vi "LoadCFG.vi"(8 "error in (no error)":errorcluster, 11 "object in":refnum<class "DIO-Configuration.lvclass">) -> (0 "error out":errorcluster, 2 "Success?":bool, 3 "object out":refnum<class "DIO-Configuration.lvclass">)   [LabVIEW 2021, in "DIO-Configuration.lvclass"]
doc: "Loads Configuration"
uses:
  DIO-Configuration.lvclass
  C:/Users/averna/Documents/LV Gym DEMO/Factory Pattern/Generic Channel/Configuration/Configuration.lvclass
  Device Channels/DAQmx/DIO-Configuration_class/tdef/Direction.ctl
  DIO-Configuration.lvclass/DIO-Configuration.ctl
  Generic Channel/Configuration/properties/ReadConfigurationFile.vi
  <vilib>/Utility/config.llb/Read Key (String).vi
  Channels/DIO-Channel/DIO-Configuration_class/DIO-Configuration.lvclass
  <vilib>/Utility/config.llb/NI_LVConfig.lvlib
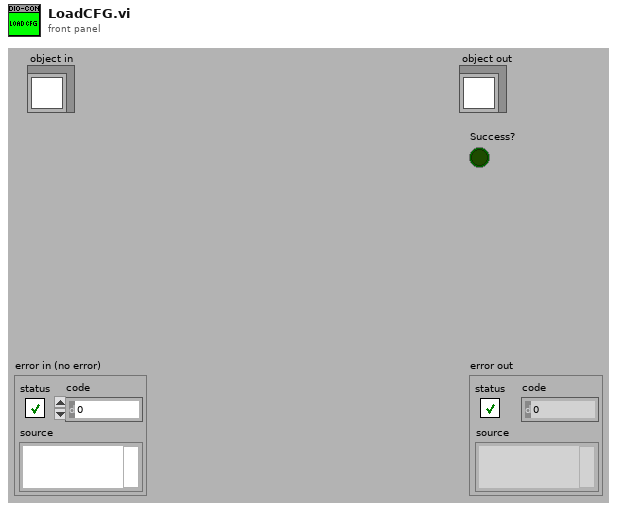
[diagram p1: front panel]
types:
  T1 = typedef "DIO-Configuration.lvclass/Direction.ctl" = enum16{"Input", "Output"}
  T2 = typedef "NI_LVConfig.lvlib/Config Data RefNum.ctl" = refnum<k1>
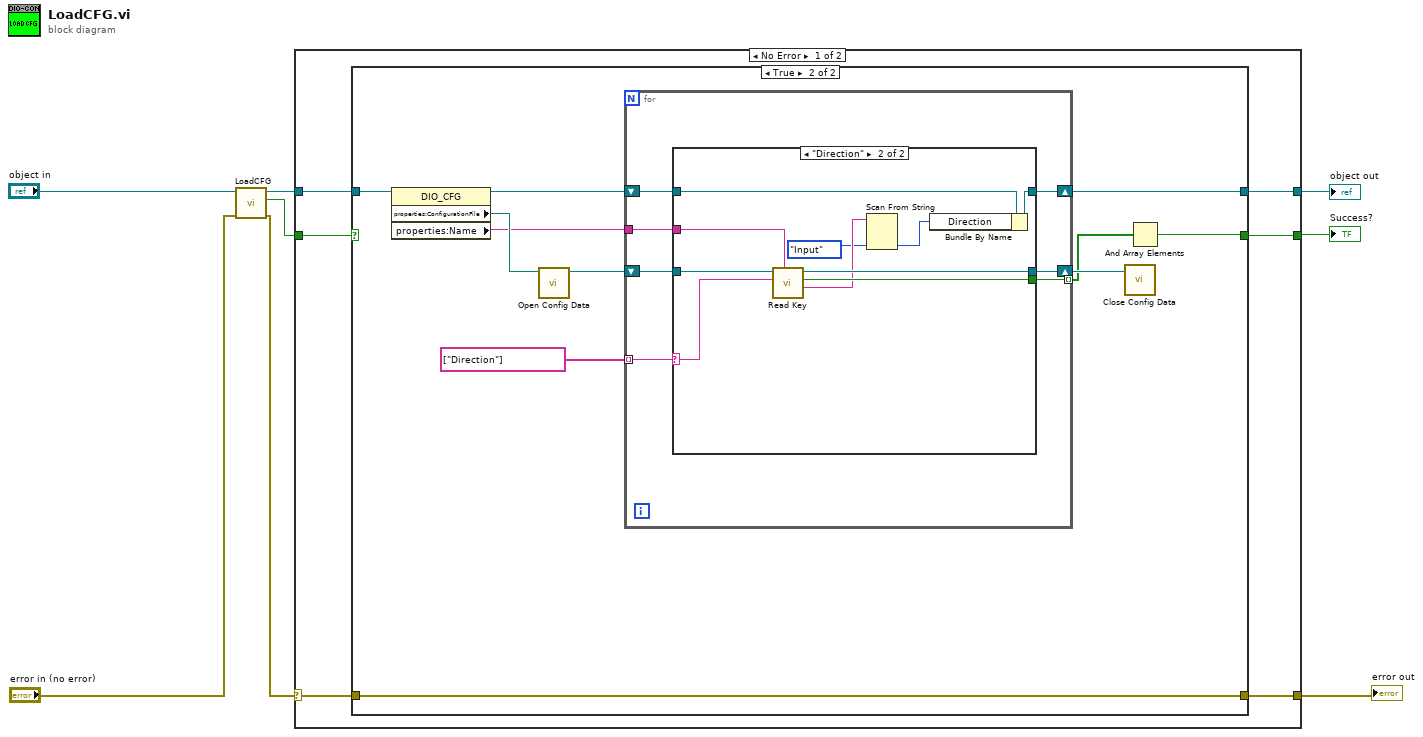
[diagram p0: block diagram]
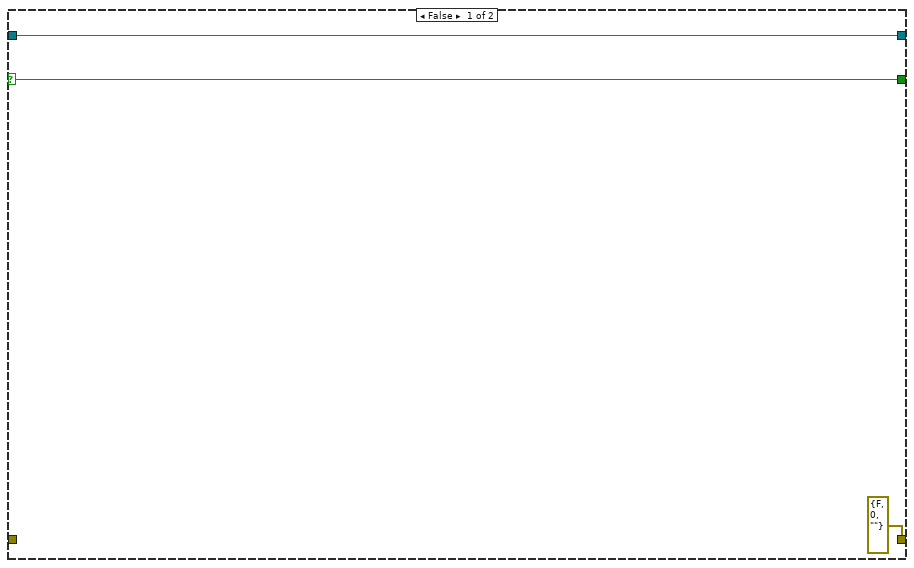
[diagram p2: hidden frame]
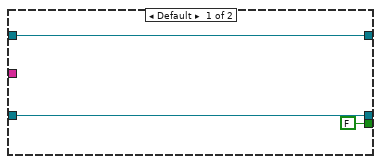
[diagram p3: hidden frame]
diagram:
  n1 = call-parent "LoadCFG.vi"("error in (no error)"="error in (no error)", "object in"="object in") -> ("error out"=w5:errorcluster, "Success?"=w3:bool, "object out"=w4:refnum<class "DIO-Configuration.lvclass">)  [unwired: 7 in]
  n2 = case shown="No Error" w5 {
    selector: w5 -> [w11 w51]
    tunnel: [w12 w51] -> w6
    tunnel: w4 -> [w13 w50]
    tunnel: [w9 w49] -> w1
    tunnel: w3 -> [w10 w49]
    tunnel: [w14 w50] -> w2
    frame No Error {
      n3 = case shown="True" w10 {
        selector: w10 -> [w16 _]
        tunnel: [w17 w24] -> w14
        tunnel: w13 -> [w17 w28]
        tunnel: [errorcluster {"status"=FALSE, "code"=0, "source"=""} ("error IO") w27] -> w12
        tunnel: w11 -> [_ w27]
        tunnel: [w16 w18] -> w9
        frame False {
        }
        frame True {
          n4 = property class="DIO_CFG"(reference=w28) -> (reference out=w23:refnum<class "DIO-Configuration.lvclass">, "properties:ConfigurationFile"=w26:path, "properties:Name"=w20:string)  [unwired: 1 in, 1 out]
          n5 = call <vilib>:"Open Config Data.vi"("configuration file path"=w26) -> ("refnum"=w25:T2)  [unwired: 8 in, 2 out]
          n6 = for {
            shift-right: [w31] -> w24
            shift-left: w23 -> [w30]
            shift-right: [w34] -> w22
            shift-left: w25 -> [w35]
            tunnel: string[] ["Direction"] -> [w33] mode=indexing
            tunnel: w20 -> [w32]
            tunnel: [w29] -> w19 mode=indexing
            n7 = case shown="\"Direction\"" w33 {
              selector: w33 -> [_ w46]
              tunnel: w35 -> [w37 w48]
              tunnel: [w37 w47] -> w34
              tunnel: w32 -> [_ w45]
              tunnel: [w38 w42] -> w31
              tunnel: w30 -> [w38 w44]
              tunnel: [FALSE ("found?") w43] -> w29
              frame Default {
              }
              frame "Direction" {
                n8 = call-poly <vilib>:"Read Key.vi"("section"=w45, "key"=w46, "refnum"=w48) -> ("value"=w41:string, "found?"=w43:bool, "refnum out"=w47:T2)  [unwired: 5 in, 1 out]
                n9 = Scan From String(input string=w41, default 1=Direction."Input" ("Data.Direction")) -> (output 1=w39:T1)  [unwired: 3 in, 3 out]
                n10 = Bundle By Name(cluster=w44, "Direction"=w39) -> (w42:refnum<class "DIO-Configuration.lvclass">)
              }
            }
          }
          n11 = call <vilib>:"Close Config Data.vi"("refnum"=w22) -> ()  [unwired: 9 in, 2 out]
          n12 = And Array Elements(Boolean array=w19) -> (logical AND=w18:bool)
        }
      }
    }
    frame Error {
    }
  }
  "error out" <- w6
  "object out" <- w2
  "Success?" <- w1
